vi "rev stat5.vi"() -> ()   [LabVIEW 2027]
uses:
  <vilib>/REVLibDriver/REVLibDriver.lvlib
  lib/libREVLibDriver.so
  <vilib>/REV Custom Controls/c_Spark_PeriodicStatus5.ctl
panel:
  out "arg2":T1
  in  "stop":bool
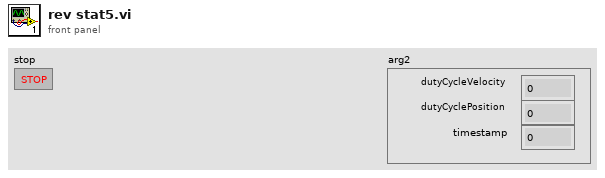
[diagram p1: front panel]
types:
  T1 = typedef "REVLibDriver.lvlib/c_Spark_PeriodicStatus5.ctl" = cluster{"dutyCycleVelocity":sgl, "dutyCyclePosition":sgl, "timestamp":u64}
  T2 = typedef "REVLibDriver.lvlib/REVSparkRefnum.ctl" = refnum<k20>
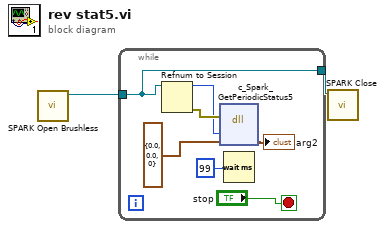
[diagram p0: block diagram]
diagram:
  n1 = call <vilib>:"SPARK Open Brushless.vi"() -> ("Spark refnum"=w2:T2)  [unwired: 10 in, 1 out]
  n2 = while {
    tunnel: w2 -> [w5]
    tunnel: [w5] -> w1
    stop <- "stop" stop-if-true
    n3 = Refnum to Session(7:w5) -> (0:w9:errorcluster, 3:w8:u64)  [unwired: 1 in]
    n4 = dll-call lib="home/systemcore/natinst/lib/libREVLibDriver.so" fn="c_Spark_GetPeriodicStatus5"(error in=w9, "hdl"=w8, "arg2"=T1 {"dutyCycleVelocity"=0.0, "dutyCyclePosition"=0.0, "timestamp"=0} ("c_Spark_PeriodicStatus5")) -> ("arg2"=→"arg2":T1)  [unwired: 4 in, 2 out]
    n5 = Wait (ms)(milliseconds to wait=u32 99) -> ()  [unwired: 1 out]
  }
  n6 = call <vilib>:"SPARK Close.vi"("Spark refnum"=w1) -> ()  [unwired: 10 in, 1 out]
